vi "Flatten .NET Symbol Information.vi"(9 "error in (no error)":errorcluster, 10 ".NET Symbol Information":refnum<k24>) -> (1 "error out":errorcluster, 2 "[.NET Symbol Information]":refnum<k24>[](array[refnum]))   [LabVIEW 2018]
uses:
  TwinCAT.Ads
  TwinCAT ADS.lvclass
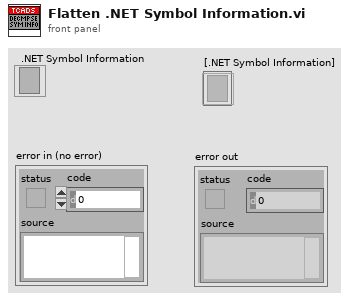
[diagram p1: front panel]
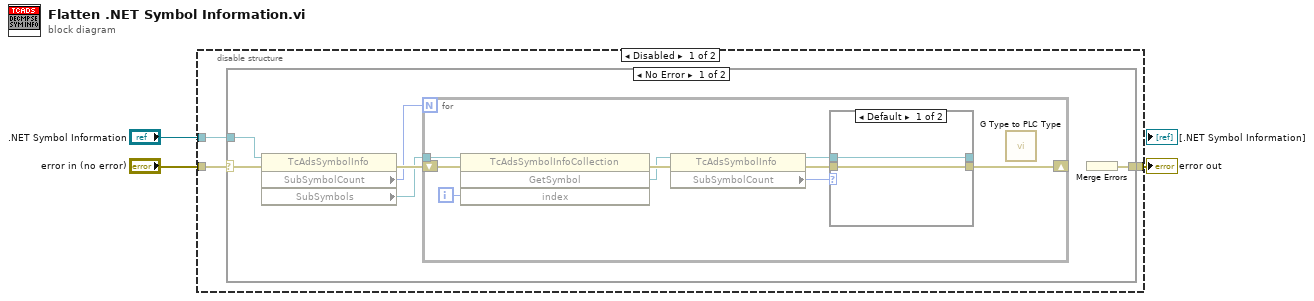
[diagram p0: block diagram]
diagram:
  n1 = disable-structure shown="Disabled" {
    disable-tunnel: "error in (no error)" -> [w6 _]
    disable-tunnel: [w5 _] -> w2
    disable-tunnel: ".NET Symbol Information" -> [w4 _]
    frame Disabled {
      n2 = case shown="No Error" w6 {
        selector: w6 -> [w10 w24]
        tunnel: [w12 w24] -> w5
        tunnel: w4 -> [w9 _]
        frame No Error {
          n3 = property class="TcAdsSymbolInfo"(reference=w9, error in=w10) -> (error out=w11:errorcluster, "SubSymbolCount"=w8:i32, "SubSymbols"=w7:refnum<k24>)  [unwired: 1 out]
          n4 = for {
            N: w8 -> [_]
            tunnel: w7 -> [w19]
            shift-right: [w13] -> _
            shift-left: w11 -> [w21]
            i -> [w20]
            n5 = invoke class="TcAdsSymbolInfoCollection" method="GetSymbol"(reference=w19, error in=w21, "index"=w20) -> (error out=w18:errorcluster, "GetSymbol"=w17:refnum<k24>)  [unwired: 1 in, 2 out]
            n6 = property class="TcAdsSymbolInfo"(reference=w17, error in=w18) -> (reference out=w14:refnum<k24>, error out=w15:errorcluster, "SubSymbolCount"=w16:i32)
            n7 = case shown="Default" w16 {
              tunnel: w15 -> [w23 _]
              tunnel: w14 -> [w22 _]
              tunnel: [w23 _] -> w13
              tunnel: [w22 _] -> _
              frame Default {
              }
              frame 0 {
              }
            }
            n8 = call "G Type to PLC Type.vi"() -> ()  [unwired: 10 in, 2 out]
          }
          n9 = Merge Errors() -> (w12:errorcluster)  [unwired: 1 in]
        }
        frame Error {
        }
      }
    }
    frame Enabled {
    }
  }
  "error out" <- w2
